vi "Write DAT (2D).vi"(4 "Append (0=F)":i32, 6 "Comments":string, 8 "error in":errorcluster, 9 "Data":dbl[][](array[numeric]), 10 "Headers":string[](array[string]), 11 "path":path) -> (0 "error out":errorcluster, 3 "new file path":path)   [LabVIEW 2019, in "LV-Data.DAT.lvclass"]
uses:
  LV-Data.DAT.lvclass
  <vilib>/Utility/file.llb/Write Delimited Spreadsheet (DBL).vi
  <vilib>/Utility/file.llb/Write Delimited Spreadsheet (string).vi
panel:
  out "appended array":string[][](array[string])
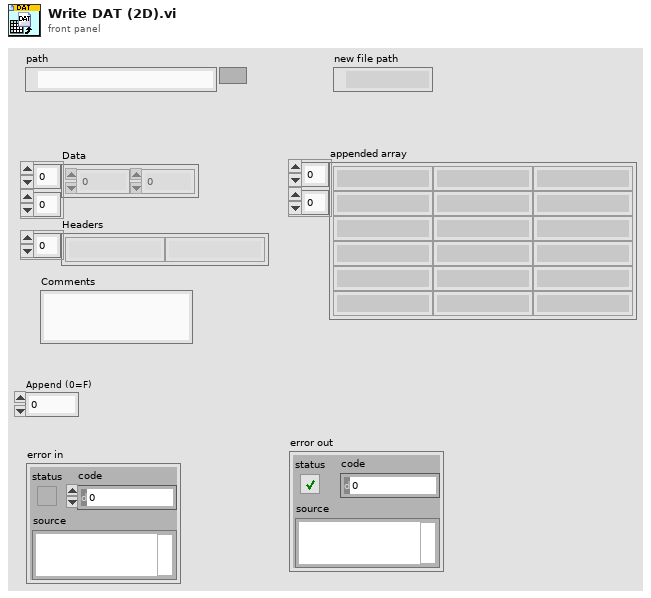
[diagram p1: front panel]
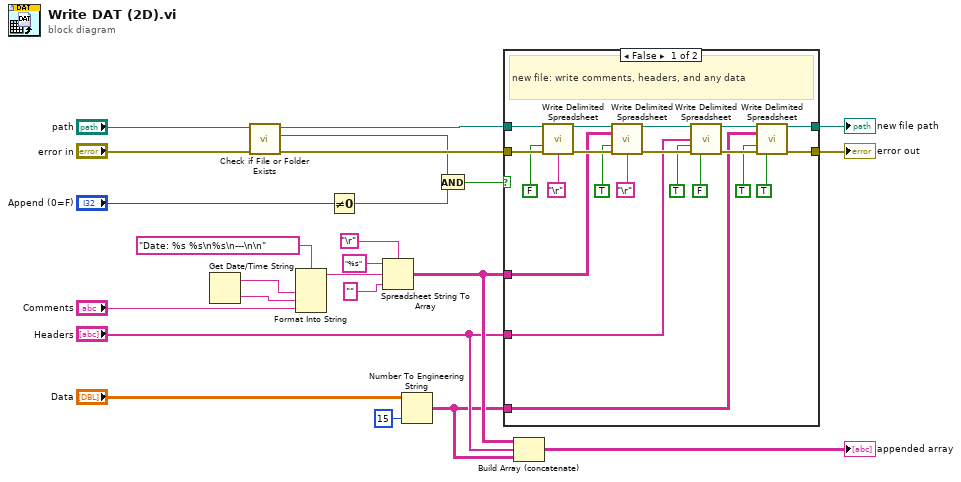
[diagram p0: block diagram]
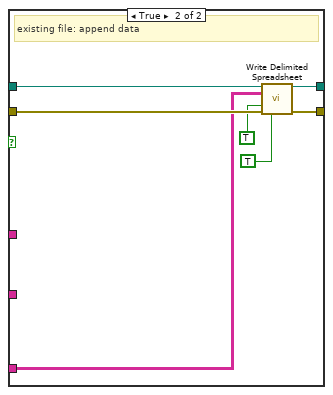
[diagram p2: hidden frame]
diagram:
  n1 = Get Date/Time String() -> (date string=w1:string, time string=w4:string)  [unwired: 3 out]
  n2 = call <vilib>:"Check if File or Folder Exists.vi"("error in (no error)"="error in", "path"="path") -> ("error out"=w10:errorcluster, "file or folder exists?"=w8:bool, "dup path"=w9:path)  [unwired: 7 in]
  n3 = Format Into String(format string="Date: %s %s\n%s\n---\n\n", w1, w4, "Comments") -> (resulting string=w2:string)  [unwired: 2 in, 1 out]
  n4 = Not Equal To 0?(x="Append (0=F)") -> (x != 0?=w7:bool)
  n5 = Spreadsheet String To Array(delimiter (Tab)="\r", format string="%s", spreadsheet string=w2, array type (2D Dbl)="") -> (array=w16:string[][])
  n6 = Number To Engineering String(2:i16 15 ("precision (6)"), 4:"Data") -> (0:w14:string[][])  [unwired: 2 out]
  n7 = And(x=w8, y=w7) -> (x .and. y?=w6:bool)
  n8 = case shown="False" w6 {
    tunnel: [w40 w50] -> w18
    tunnel: w9 -> [w45 w52]
    tunnel: w10 -> [w44 w51]
    tunnel: [w41 w49] -> w19
    tunnel: w14 -> [w33 w48]
    tunnel: "Headers" -> [w34 _]
    tunnel: w16 -> [w35 _]
    frame False {
      # "new file: write comments, headers, and any data"
      n9 = call-poly <vilib>:"Write Delimited Spreadsheet.vi"("file path (dialog if empty)"=w45, "append to file? (new file:F)"=FALSE, "error in (no error)"=w44, "delimiter (\\t)"="\r") -> ("new file path (Not A Path if cancelled)"=w38:path, "error out"=w39:errorcluster)  [unwired: 10 in]
      n10 = call-poly <vilib>:"Write Delimited Spreadsheet.vi"("file path (dialog if empty)"=w38, "2D data"=w35, "append to file? (new file:F)"=TRUE, "error in (no error)"=w39, "delimiter (\\t)"="\r") -> ("new file path (Not A Path if cancelled)"=w37:path, "error out"=w36:errorcluster)  [unwired: 9 in]
      n11 = call-poly <vilib>:"Write Delimited Spreadsheet.vi"("file path (dialog if empty)"=w37, "1D data"=w34, "append to file? (new file:F)"=TRUE, "error in (no error)"=w36, "transpose? (no:F)"=FALSE) -> ("new file path (Not A Path if cancelled)"=w42:path, "error out"=w43:errorcluster)  [unwired: 9 in]
      n12 = call-poly <vilib>:"Write Delimited Spreadsheet.vi"("file path (dialog if empty)"=w42, "2D data"=w33, "append to file? (new file:F)"=TRUE, "error in (no error)"=w43, "transpose? (no:F)"=TRUE) -> ("new file path (Not A Path if cancelled)"=w40:path, "error out"=w41:errorcluster)  [unwired: 9 in]
    }
    frame True {
      # "existing file: append data"
      n13 = call-poly <vilib>:"Write Delimited Spreadsheet.vi"("file path (dialog if empty)"=w52, "2D data"=w48, "append to file? (new file:F)"=TRUE, "error in (no error)"=w51, "transpose? (no:F)"=TRUE) -> ("new file path (Not A Path if cancelled)"=w50:path, "error out"=w49:errorcluster)  [unwired: 9 in]
    }
  }
  "new file path" <- w18
  "error out" <- w19
  n14 = Build Array (concatenate)(w16, "Headers", w14) -> (→"appended array":string[][])
